vi "Plot Bezier Curve.vi"() -> ()   [LabVIEW 2020]
panel:
  out "Curve Graph 6":cluster{"position out":sgl[], "y":dbl[]}(graph)
  out "x-y 3":u32
  out "l":dbl
  out "l total":dbl
  out "Array 3":sgl[](array[numeric])
  out "Curve Graph 3":cluster{sgl, sgl}[](graph)
  out "Curve Graph 2":cluster{sgl, sgl}[](graph)
  out "Curvature":dbl[](graph)
  out "appended array":cluster{"x":dbl, "y":dbl}[](array[cluster])
  out "d2 ctrl pts":cluster{dbl, dbl}[](array[cluster])
  out "2nd derivative":cluster{"x":sgl, "y":sgl}[](graph)
  out "1st derivative":cluster{"x":sgl, "y":sgl}[](graph)
  out "d ctrl pts":cluster{dbl, dbl}[](array[cluster])
  out "size(s)":i32
  out "Curve Graph":cluster{"x":sgl, "y":sgl}[](graph)
  out "x-y":u32
  in  "percision":dbl=0.01
  in  "ctrl points":cluster{dbl, dbl}[](array[cluster])
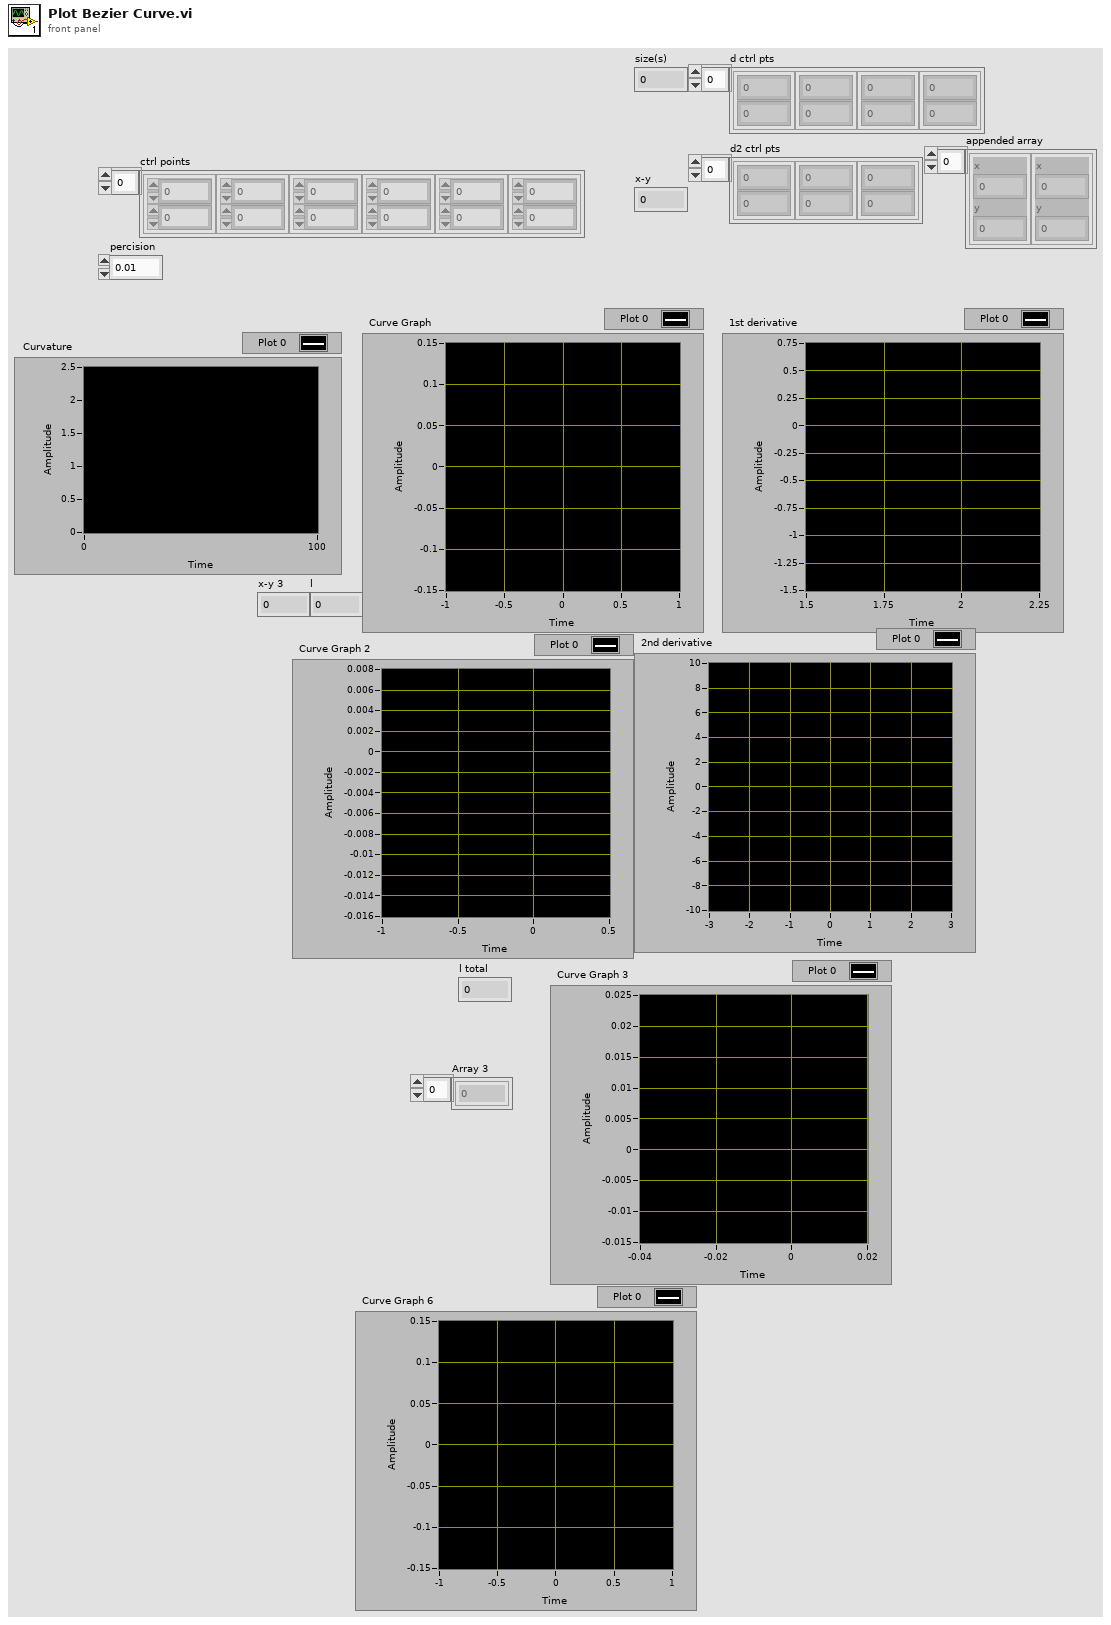
[diagram p1: front panel]
types:
  T1 = typedef "Bezier Curve.ctl" = cluster{"x":sgl, "y":sgl}[]
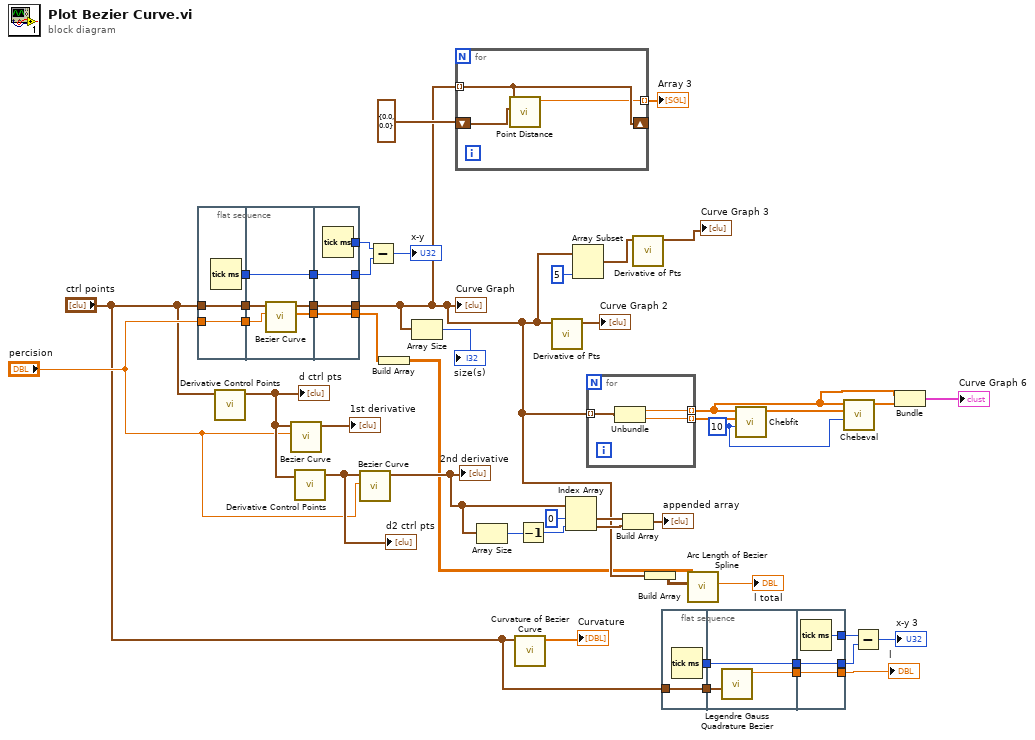
[diagram p0: block diagram]
diagram:
  w1 = u16 10 ("degree")
  n1 = flat-sequence {
    tunnel: "percision" -> [w50]
    tunnel: "ctrl points" -> [w51]
    tunnel: [w51] -> w47
    tunnel: [w50] -> w46
    tunnel: [w49] -> w42
    tunnel: [w53] -> w48
    tunnel: w47 -> [w56]
    tunnel: w46 -> [w54]
    tunnel: [w55] -> w43
    tunnel: w42 -> [w55]
    tunnel: [w52] -> w9
    tunnel: [w60] -> w11
    tunnel: w48 -> [w60]
    tunnel: [w59] -> w45
    tunnel: [w58] -> w44
    tunnel: w43 -> [w58]
    tunnel: [w57] -> w3
    tunnel: w9 -> [w57]
    frame #0 {
      n2 = Tick Count (ms)() -> (millisecond timer value=w49:u32)
    }
    frame #1 {
      n3 = call "Bezier Curve.vi"("percision"=w54, "ctrl points"=w56) -> ("position out"=w52:sgl[], "curve"=w53:T1)  [unwired: 8 in]
    }
    frame #2 {
      n4 = Tick Count (ms)() -> (millisecond timer value=w59:u32)
    }
  }
  n5 = call "Derivative Control Points.vi"("ctrl points"="ctrl points") -> ("d ctrl pts"=w38:cluster{dbl, dbl}[])  [unwired: 10 in]
  "d ctrl pts" <- w38
  n6 = call "Bezier Curve.vi"("percision"="percision", "ctrl points"=w38) -> ("curve"=→"1st derivative":T1)  [unwired: 8 in, 1 out]
  n7 = call "Derivative Control Points.vi"("ctrl points"=w38) -> ("d ctrl pts"=w37:cluster{dbl, dbl}[])  [unwired: 10 in]
  "d2 ctrl pts" <- w37
  n8 = call "Bezier Curve.vi"("percision"="percision", "ctrl points"=w37) -> ("curve"=w36:T1)  [unwired: 8 in, 1 out]
  "2nd derivative" <- w36
  n9 = Subtract(x=w45, y=w44) -> (x-y=→"x-y":u32)
  n10 = Build Array(w3) -> (w2:sgl[][])
  n11 = Array Size(array=w11) -> (size(s)=→"size(s)":i32)
  n12 = for {
    tunnel: w11 -> [w62] mode=indexing
    shift-right: [w62] -> _
    shift-left: cluster{"x":sgl, "y":sgl} {"x"=0.0, "y"=0.0} ("element") -> [w63]
    tunnel: [w61] -> w22 mode=indexing
    n13 = call "Point Distance.vi"("point b"=w63, "point a"=w62) -> ("dist"=w61:sgl)  [unwired: 9 in]
  }
  "Array 3" <- w22
  n14 = Array Size(array=w36) -> (size(s)=w35:i32)
  n15 = call "Curvature of Bezier Curve.vi"("curve"="ctrl points") -> ("curvature"=→"Curvature":dbl[])  [unwired: 10 in]
  n16 = Decrement(x=w35) -> (x-1=w34:i32)
  n17 = call "Derivative of Pts.vi"("pts"=w11) -> ("pts out"=→"Curve Graph 2":cluster{sgl, sgl}[])  [unwired: 10 in]
  n18 = Index Array(array=w36, index #1=0 ("index"), index #2=w34) -> (element #1=w32:cluster{"x":sgl, "y":sgl}, element #2=w31:cluster{"x":sgl, "y":sgl})
  n19 = Array Subset(array=w11, length=5) -> (w25:T1)  [unwired: 1 in]
  n20 = for {
    tunnel: w11 -> [w66] mode=indexing
    tunnel: [w65] -> w6 mode=indexing
    tunnel: [w64] -> w10 mode=indexing
    n21 = Unbundle(w66) -> ("x"=w65:sgl, "y"=w64:sgl)
  }
  n22 = Build Array(w32, w31) -> (→"appended array":cluster{"x":sgl, "y":sgl}[])
  n23 = call "Derivative of Pts.vi"("pts"=w25) -> ("pts out"=→"Curve Graph 3":cluster{sgl, sgl}[])  [unwired: 10 in]
  n24 = Build Array(w11) -> (w4:cluster{"x":sgl, "y":sgl}[][])
  n25 = flat-sequence {
    tunnel: "ctrl points" -> [w68]
    tunnel: [w68] -> w17
    tunnel: [w67] -> w13
    tunnel: [w70] -> w18
    tunnel: w17 -> [w71]
    tunnel: [w69] -> w14
    tunnel: w13 -> [w69]
    tunnel: [w74] -> w19
    tunnel: w18 -> [w74]
    tunnel: [w73] -> w16
    tunnel: [w72] -> w15
    tunnel: w14 -> [w72]
    frame #0 {
      n26 = Tick Count (ms)() -> (millisecond timer value=w67:u32)
    }
    frame #1 {
      n27 = call "Legendre Gauss Quadrature Bezier.vi"("ctrl points"=w71) -> ("l"=w70:dbl)  [unwired: 10 in]
    }
    frame #2 {
      n28 = Tick Count (ms)() -> (millisecond timer value=w73:u32)
    }
  }
  n29 = call "Arc Length of Bezier Spline.vi"("ctrl pts"=w4, "position"=w2) -> ("l total"=→"l total":dbl)  [unwired: 6 in, 3 out]
  n30 = call "Chebfit.vi"("degree"=w1, "Y"=w10, "X"=w6) -> ("C"=w5:dbl[])  [unwired: 8 in]
  n31 = call "Chebeval.vi"("degree"=w1, "Cheby weights"=w5, "x"=w6) -> ("y"=w8:dbl[])  [unwired: 8 in]
  n32 = Subtract(x=w16, y=w15) -> (x-y=→"x-y 3":u32)
  n33 = Bundle(w6, "y"=w8) -> (→"Curve Graph 6":cluster{sgl[], "y":dbl[]})  [unwired: 1 in]
  "Curve Graph" <- w11
  "l" <- w19
